vi "mupDefineVar_Array.vi"(8 "error in (no error)":errorcluster, 9 "initValue":dbl[](array[numeric]), 10 "varName":string, 11 "hParser in":u64) -> (0 "error out":errorcluster, 2 "varAddr":u64, 3 "hParser out":u64)   [LabVIEW 2018, in "mupLib.lvlib"]
doc: "Define a variable and set its initial values for bulk mode evaluation.\nThe variable's pointer is returned in varAddr."
uses:
  mupLib.lvlib
  <vilib>/Utility/error.llb/Error Cluster From Error Code.vi
  libmuparser-lv.dll
panel:
  # "Define a variable and set its initial values for bulk mode evaluation.\nThe variable's pointer is returned in varAddr."
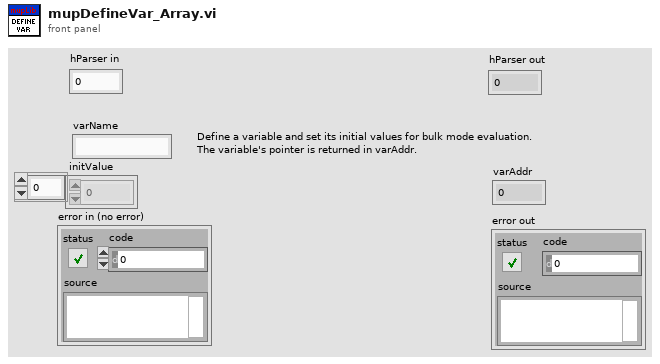
[diagram p1: front panel]
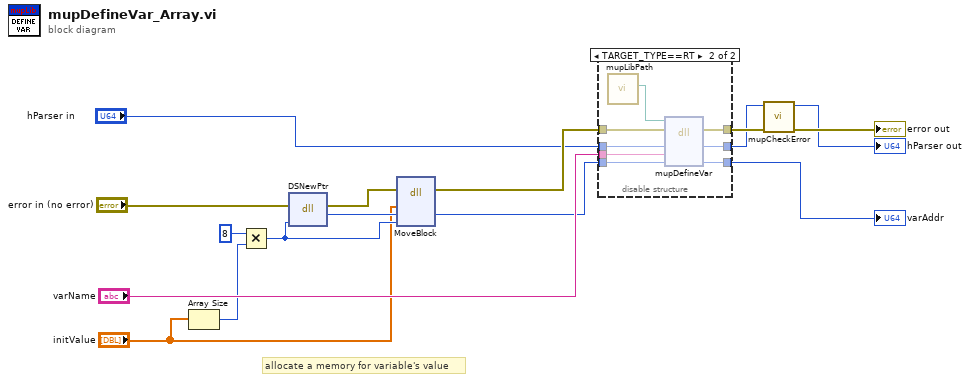
[diagram p0: block diagram]
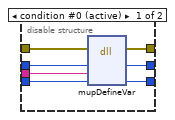
[diagram p2: hidden frame]
diagram:
  # "allocate a memory for variable's value"
  n1 = Array Size(array="initValue") -> (size(s)=w1:i32)
  n2 = Multiply(x=8 ("size"), y=w1) -> (x*y=w3:i32)
  n3 = dll-call lib="LabVIEW" fn="DSNewPtr"(error in="error in (no error)", "size"=w3) -> (error out=w15:errorcluster, "return type"=w16:u64)  [unwired: 3 in, 1 out]
  n4 = dll-call lib="LabVIEW" fn="MoveBlock"(error in=w15, "ps"="initValue", "pd"=w16, "size"=w3) -> (error out=w14:errorcluster, "pd"=w12:u64)  [unwired: 5 in, 1 out]
  n5 = disable-structure shown="TARGET_TYPE==RT" {
    disable-tunnel: w14 -> [w23 w31]
    disable-tunnel: "varName" -> [w22 w30]
    disable-tunnel: w12 -> [w21 w29]
    disable-tunnel: [w20 w28] -> w11
    disable-tunnel: [w19 w27] -> w9
    disable-tunnel: "hParser in" -> [w18 w26]
    disable-tunnel: [w17 w25] -> w5
    frame condition #0 (active) {
      n6 = dll-call lib="C:/Users/leonidas/Documents/GitHub/LV-muParser/mupLib/libmuparser-lv.dll" fn="mupDefineVar"(error in=w23, "hParser"=w18, "szName"=w22, "fVar"=w21) -> (error out=w19:errorcluster, "hParser"=w17:u64, "fVar"=w20:u64)  [unwired: 4 in, 1 out]
    }
    frame condition #1 {
      n7 = call "mupLibPath.vi"() -> ("libmuparser path"=w24:path)  [unwired: 11 in]
      n8 = dll-call lib="C:/Users/leonidas/Documents/GitHub/LV-muParser/mupLib/libmuparser-lv.dll" fn="mupDefineVar"(path in=w24, error in=w31, "hParser"=w26, "szName"=w30, "fVar"=w29) -> (error out=w27:errorcluster, "hParser"=w25:u64, "fVar"=w28:u64)  [unwired: 3 in, 1 out]
    }
  }
  "varAddr" <- w11
  n9 = call "mupCheckError.vi"("error in (no error)"=w9, "hParser in"=w5) -> ("error out"=→"error out":errorcluster, "hParser out"=→"hParser out":u64)  [unwired: 8 in]
